vi "Create.vi"(8 "error in (no error)":errorcluster) -> (0 "error out":errorcluster, 3 "Client out":refnum<class "Client.lvclass">)   [LabVIEW 2020, in "PV Access.lvlib" / "PVA Client.lvlib" / "Client.lvclass"]
doc: "Create a new client."
uses:
  Client.lvclass
  PV Access.lvlib
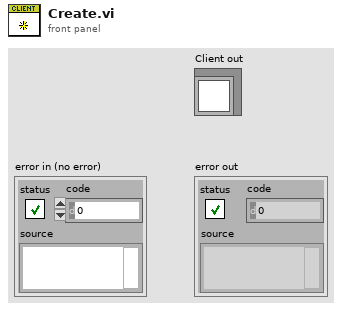
[diagram p1: front panel]
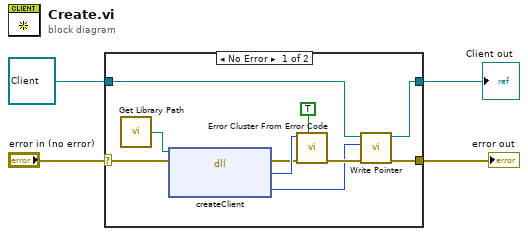
[diagram p0: block diagram]
diagram:
  n1 = case shown="No Error" "error in (no error)" {
    selector: "error in (no error)" -> [w14 w16]
    tunnel: [w8 w16] -> w3
    tunnel: [w6 w15] -> w1
    tunnel: refnum<class "Client.lvclass"> refnum ("Client in") -> [w7 w15]
    frame No Error {
      n2 = call "Get Library Path.vi"() -> ("Path"=w11:path)  [unwired: 1 in]
      n3 = dll-call lib="?" fn="createClient"(path in=w11, error in=w14) -> (error out=w12:errorcluster, "ret_code"=w13:i32, "client"=w5:i64)  [unwired: 2 in, 1 out]
      n4 = call <vilib>:"Error Cluster From Error Code.vi"("show call chain? (False)"=TRUE, "error in (no error)"=w12, "error code (0)"=w13) -> ("error out"=w9:errorcluster)  [unwired: 6 in]
      n5 = call-dynamic "Write Pointer.vi"("error in (no error)"=w9, "Pointer"=w5, "Pointer Base in"=w7) -> ("error out"=w8:errorcluster, "Pointer Base out"=w6:refnum<class "Client.lvclass">)  [unwired: 7 in]
    }
    frame Error {
    }
  }
  "error out" <- w3
  "Client out" <- w1
